vi "Connect 3D Controller.vi"(8 "error in (no error)":errorcluster caption="에러 입력(에러 없음)", 10 "VISA resource name":refnum<visa-resource-name>, 11 "Instrument Manager 입력":refnum<class "Instrument Manager.lvclass">) -> (0 "error out":errorcluster caption="에러 출력", 2 "Connected?":bool, 3 "Instrument Manager 출력":refnum<class "Instrument Manager.lvclass">)   [LabVIEW 2023, in "Instrument Manager.lvclass"]
uses:
  Instrument Manager.lvclass
  Instrument Manager.lvclass/Instrument Manager.ctl
  Module/FCC FR2 3D Controller Module/3D Controller/3D Controller.lvclass
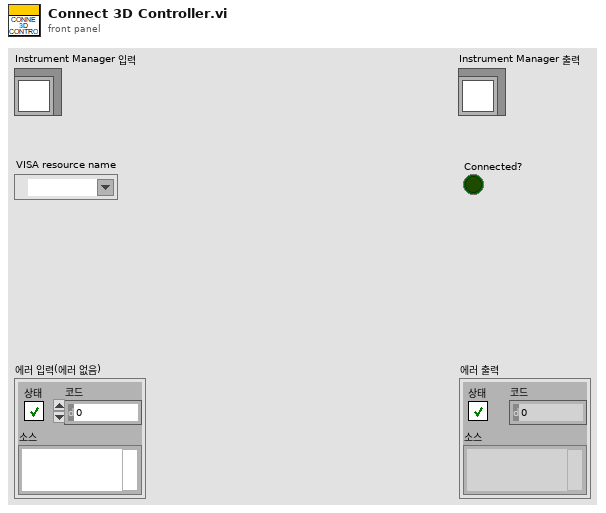
[diagram p1: front panel]
types:
  T1 = cluster{"Anritsu Call Box":refnum<class "Anritsu Call Box.lvclass">, "Spectrum Analyzer":refnum<class "Interface_Spectrum.lvclass">, "RF Switch Box":refnum<class "RF Filter Box.lvclass">, "Turn Table":refnum<class "Interface - Turn Table.lvclass">, "Mast":refnum<class "Interface - Mast.lvclass">, "3D Controller":refnum<class "Interface_3D Controller.lvclass">}
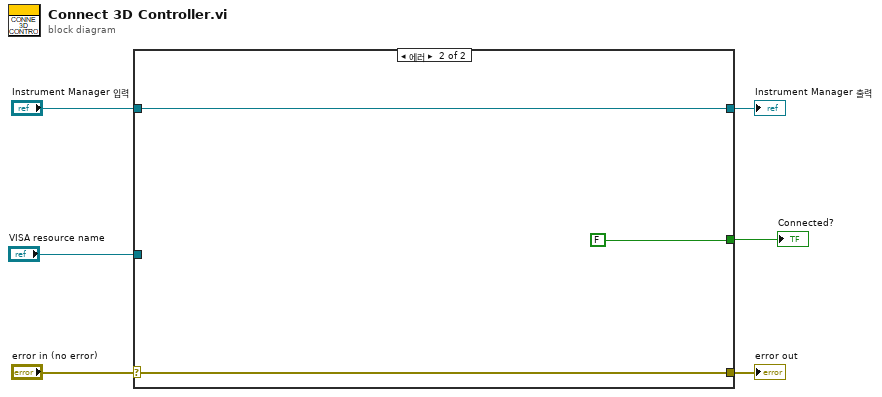
[diagram p0: block diagram]
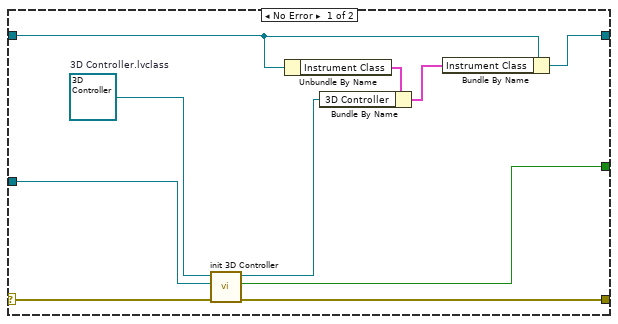
[diagram p2: hidden frame]
diagram:
  n1 = case shown="에러" "error in (no error)" {
    selector: "error in (no error)" -> [w11 w19]
    tunnel: [w10 w19] -> w5
    tunnel: [w13 w18] -> w3
    tunnel: "Instrument Manager 입력" -> [w15 w18]
    tunnel: "VISA resource name" -> [w9 _]
    tunnel: [w7 FALSE ("Connected?")] -> w1
    frame No Error {
      w16 = refnum<class "3D Controller.lvclass"> refnum  # 3D Controller.lvclass
      n2 = call-dynamic "init 3D Controller.vi"("error in (no error)"=w11, "VISA resource name"=w9, "3D Controller in"=w16) -> ("error out"=w10:errorcluster, "Connected?"=w7:bool, "3D Controller out"=w8:refnum<class "3D Controller.lvclass">)  [unwired: 6 in]
      n3 = Unbundle By Name(w15) -> ("Instrument Class"=w14:T1)
      n4 = Bundle By Name(cluster=w14, "3D Controller"=w8) -> (w12:T1)
      n5 = Bundle By Name(cluster=w15, "Instrument Class"=w12) -> (w13:refnum<class "Instrument Manager.lvclass">)
    }
    frame Error {
    }
  }
  "error out" <- w5
  "Instrument Manager 출력" <- w3
  "Connected?" <- w1
